vi "Build VIH Deploy - Create Project.vi"(8 "error in":errorcluster, 10 "Project Files":path[](array[path]), 11 "Target Dir":path) -> (0 "error out":errorcluster, 2 "Project File Path":path, 3 "dup Target Dir":path)   [LabVIEW 2014]
doc: "::: VI Helpeks :::\nCopyright (c) 2000-2026 Konstantin Shifershteyn. All rights reserved."
panel:
  # "VI Helpeks\nCopyright (c) 2012-2026 Konstantin Shifershteyn"
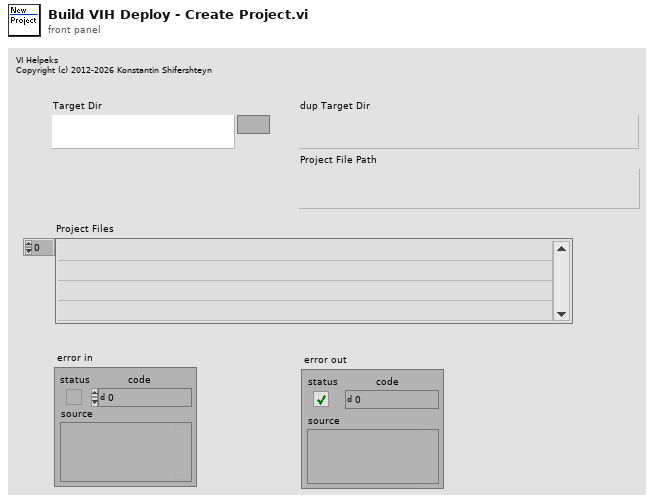
[diagram p1: front panel]
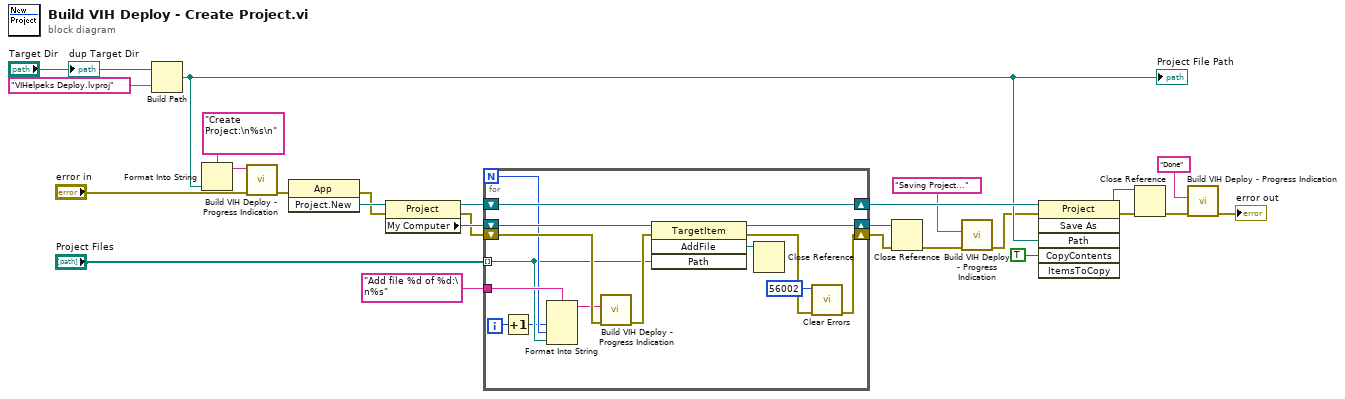
[diagram p0: block diagram]
diagram:
  n1 = Build Path(base path="Target Dir", name or relative path="VIHelpeks Deploy.lvproj") -> (appended path=w7:path)
  "Project File Path" <- w7
  n2 = Format Into String(format string="Create Project:\n%s\n", w7) -> (resulting string=w9:string)  [unwired: 2 in, 1 out]
  n3 = call "Build VIH Deploy - Progress Indication.vi"("error in"="error in", "message 1"=w9) -> ("error out"=w11:errorcluster)  [unwired: 9 in]
  n4 = invoke class="App" method="Project.New"(error in=w11) -> (error out=w22:errorcluster, "Project:New"=w24:refnum<vi>)  [unwired: 2 in, 1 out]
  n5 = property class="Project"(reference=w24, error in=w22) -> (reference out=w26:refnum<vi>, error out=w20:errorcluster, "My Computer"=w23:refnum<vi>)
  n6 = for {
    N -> [w33]
    tunnel: "Project Files" -> [w32] mode=indexing
    shift-right: [w40] -> w21
    shift-left: w23 -> [w41]
    shift-right: [w27] -> w25
    shift-left: w20 -> [w37]
    shift-right: [w38] -> w14
    shift-left: w26 -> [w38]
    tunnel: "Add file %d of %d:\n%s" -> [w35]
    i -> [w34]
    n7 = Increment(x=w34) -> (x+1=w31:i32)
    n8 = Format Into String(format string=w35, w31, w33, w32) -> (resulting string=w30:string)  [unwired: 2 in, 1 out]
    n9 = call "Build VIH Deploy - Progress Indication.vi"("error in"=w37, "message 2"=w30) -> ("error out"=w36:errorcluster)  [unwired: 9 in]
    n10 = invoke class="TargetItem" method="AddFile"(reference=w41, error in=w36, "Path"=w32) -> (reference out=w40:refnum<vi>, error out=w28:errorcluster, "AddFile"=w39:refnum<vi>)  [unwired: 1 in, 1 out]
    n11 = Close Reference(reference=w39) -> ()  [unwired: 1 in, 1 out]
    n12 = call <vilib>:"Clear Errors.vi"("error in (no error)"=w28, "specific error code to clear (0: all)"=56002) -> ("error out"=w27:errorcluster)  [unwired: 4 in, 1 out]
  }
  n13 = Close Reference(reference=w21, error in (no error)=w25) -> (error out=w6:errorcluster)
  n14 = call "Build VIH Deploy - Progress Indication.vi"("error in"=w6, "message 2"="Saving Project...") -> ("error out"=w5:errorcluster)  [unwired: 9 in]
  n15 = invoke class="Project" method="Save As"(reference=w14, error in=w5, "Path"=w7, "CopyContents"=TRUE ("Copy contents?")) -> (reference out=w17:refnum<vi>, error out=w18:errorcluster)  [unwired: 2 in, 4 out]
  n16 = Close Reference(reference=w17, error in (no error)=w18) -> (error out=w3:errorcluster)
  n17 = call "Build VIH Deploy - Progress Indication.vi"("error in"=w3, "message 2"="Done") -> ("error out"=→"error out":errorcluster)  [unwired: 9 in]
  "dup Target Dir" <- "Target Dir"
